vi "InitModuleManager.vi"(8 "error in (no error)":errorcluster, 10 "mmanager":path, 11 "SensorInfos":T3) -> (0 "error out (no error)":errorcluster, 3 "Sensor Engine Datas":T1[](array[typedef]))   [LabVIEW 2023, in "MM.lvlib"]
uses:
  MM.lvlib
  Shared/SensorInfos.ctl
  Shared/SensorInfo.ctl
  Shared/Sensor Name.ctl
  Shared/Protocol.ctl
  MM Data.ctl
  MM Objects.ctl
  MM Object.ctl
  Sensor Engine Data.ctl
  DataContainer/DataContainer.lvclass
  <vilib>/xnet/xnet.llb/XNET Frame FlexRay.ctl
  <vilib>/xnet/xnet.llb/XNET Frame Type FlexRay.ctl
  <vilib>/xnet/xnet.llb/XNET String To IO Name (Signal).vi
  <vilib>/xnet/xnet.llb/XNET Create Session (Conversion).vi
  <resource>/objmgr/xnet.rc
  Shared/Vires VTD Shared.lvlib
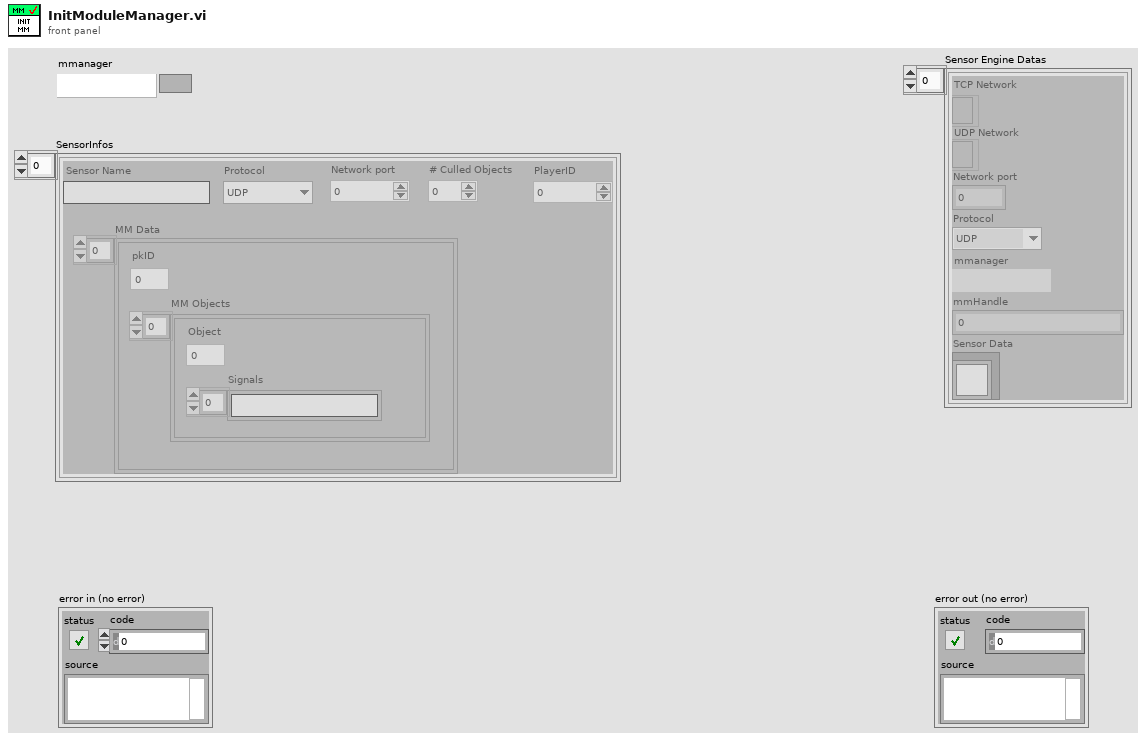
[diagram p1: front panel]
types:
  T1 = typedef "MM.lvlib/Sensor Engine Data.ctl" = cluster{"TCP Network":refnum<k5>, "UDP Network":refnum<k16>, "Network port":i32, "Protocol":T2, "mmanager":path, "mmHandle":u64, "Sensor Data":refnum<class "DataContainer.lvclass">}
  T2 = typedef "Vires VTD Shared.lvlib/Protocol.ctl" = enum16{"UDP", "TCP"}
  T3 = typedef "Vires VTD Shared.lvlib/SensorInfos.ctl" = T4[]
  T4 = typedef "Vires VTD Shared.lvlib/SensorInfo.ctl" = cluster{"Sensor Name":T5, "Protocol":T2, "Network port":i32, "# Culled Objects":i32, "PlayerID":u8, "MM Data":T6}
  T5 = typedef "Vires VTD Shared.lvlib/Sensor Name.ctl" = string
  T6 = typedef "Vires VTD Shared.lvlib/MM Data.ctl" = T7[]
  T7 = typedef "MM.lvlib/MM Objects.ctl" = cluster{"pkID":i32, "MM Objects":T8[]}
  T8 = typedef "MM.lvlib/MM Object.ctl" = cluster{"Object":i32, "Signals":string[]}
  T9 = typedef "XNET Frame FlexRay.ctl" = cluster{"timestamp":timestamp, "payload":u8[], "slot":u16, "type":T10, "cycle count":u8, "startup?":bool, "sync?":bool, "preamble?":bool, "ch A":bool, "ch B":bool, "echo?":bool}
  T10 = typedef "XNET Frame Type FlexRay.ctl" = u8
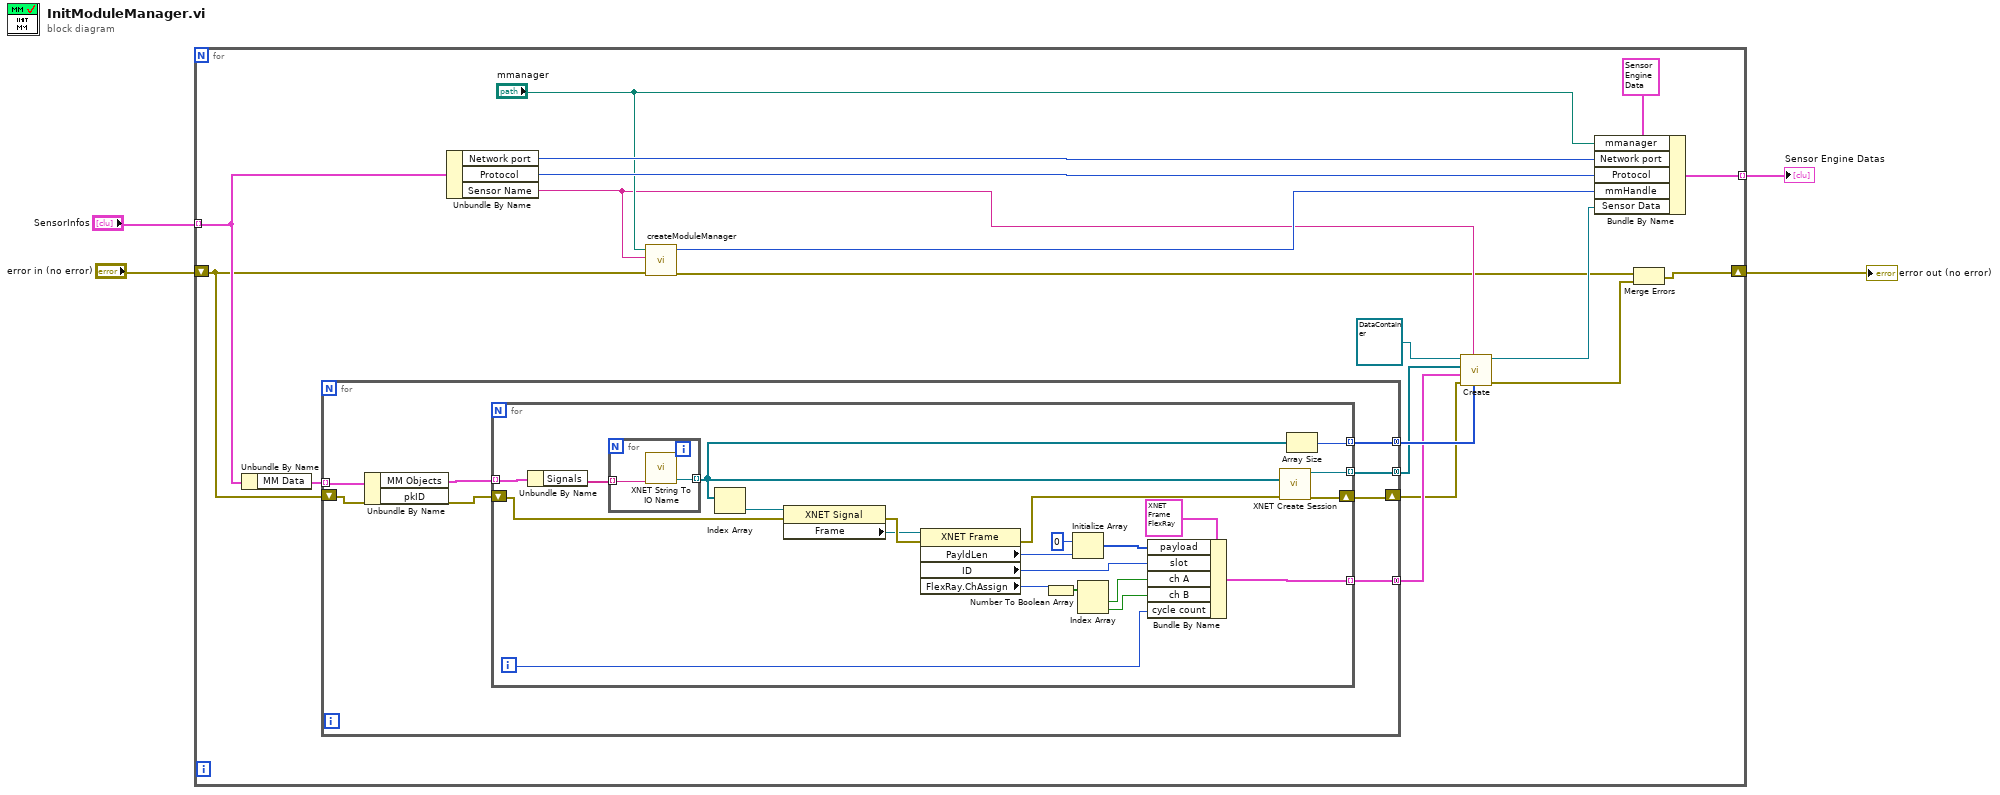
[diagram p0: block diagram]
diagram:
  n1 = for {
    tunnel: "SensorInfos" -> [w23] mode=indexing
    shift-right: [w5] -> w4
    shift-left: "error in (no error)" -> [w9]
    tunnel: [w18] -> w2 mode=indexing
    n2 = Unbundle By Name(w23) -> ("MM Data"=w22:T6)
    n3 = for {
      shift-right: [w30] -> w8
      shift-left: w9 -> [w29]
      tunnel: [w28] -> w12 mode=concatenating
      tunnel: [w27] -> w11 mode=concatenating
      tunnel: w22 -> [w26] mode=indexing
      tunnel: [w24] -> w14 mode=concatenating
      n4 = Unbundle By Name(w26) -> ("MM Objects"=w25:T8[])  [unwired: 1 out]
      n5 = for {
        tunnel: [w39] -> w27 mode=indexing
        tunnel: [w35] -> w28 mode=indexing
        shift-right: [w37] -> w30
        shift-left: w29 -> [w36]
        tunnel: w25 -> [w34] mode=indexing
        tunnel: [w31] -> w24 mode=indexing
        i -> [w33]
        n6 = Unbundle By Name(w34) -> ("Signals"=w52:string[])
        n7 = for {
          tunnel: w52 -> [w54] mode=indexing
          tunnel: [w53] -> w32 mode=indexing
          n8 = call-poly <vilib>:"XNET String To IO Name.vi"("string"=w54) -> ("XNET Signal"=w53:refnum<k21>)  [unwired: 4 out]
        }
        n9 = Index Array(array=w32) -> (element=w40:refnum<k21>)  [unwired: 1 in]
        n10 = property class="XNET Signal"(reference=w40, error in=w36) -> (error out=w51:errorcluster, "Frame"=w50:refnum<k21>)  [unwired: 1 out]
        n11 = property class="XNET Frame"(reference=w50, error in=w51) -> (error out=w38:errorcluster, "PayldLen"=w43:u32, "ID"=w45:u32, "FlexRay.ChAssign"=w46:u32)  [unwired: 1 out]
        n12 = Number To Boolean Array(number=w46) -> (Boolean array=w41:bool[])
        n13 = Initialize Array(u8 0 ("element"), w43) -> (w44:u8[])
        n14 = Index Array(array=w41) -> (element #1=w47:bool, element #2=w48:bool)  [unwired: 2 in]
        n15 = Bundle By Name(cluster=T9 {"timestamp"=timestamp(0 s since 1904-01-01), "payload"=[], "slot"=1, "type"=32, "cycle count"=0, "startup?"=FALSE, "sync?"=FALSE, "preamble?"=FALSE, "ch A"=FALSE, "ch B"=FALSE, "echo?"=FALSE} ("FlexRay frame"), "payload"=w44, "slot"=w45, "ch A"=w47, "ch B"=w48, "cycle count"=w33) -> (w39:T9)
        n16 = call-poly <vilib>:"XNET Create Session.vi"("signal list"=w32, "error in (no error)"=w38) -> ("session out"=w35:refnum<k21>, "error out"=w37:errorcluster)  [unwired: 12 in]
        n17 = Array Size(array=w32) -> (size(s)=w31:i32)
      }
    }
    n18 = Unbundle By Name(w23) -> ("Network port"=w20:i32, "Protocol"=w19:T2, "Sensor Name"=w15:T5)
    n19 = call "createModuleManager.vi"("error in (no error)"=w9, "sensorName"=w15, "path in"="mmanager") -> ("error out"=w7:errorcluster, "mmHandle"=w16:u64)  [unwired: 7 in]
    n20 = call-dynamic "Create.vi"("noSignals"=w14, "Container ID"=w15, "error in (no error)"=w8, "Package Data"=w11, "Conversion References"=w12, "DataContainer in"=refnum<class "DataContainer.lvclass"> refnum) -> ("error out"=w6:errorcluster, "DataContainer out"=w10:refnum<class "DataContainer.lvclass">)  [unwired: 4 in]
    n21 = Bundle By Name(cluster=T1 {"TCP Network"=refnum, "UDP Network"=refnum, "Network port"=0, "Protocol"=enum."UDP", "mmanager"=path "", "mmHandle"=0, "Sensor Data"=refnum} ("MM.lvlib:Sensor Engine Data"), "mmanager"="mmanager", "Network port"=w20, "Protocol"=w19, "mmHandle"=w16, "Sensor Data"=w10) -> (w18:T1)
    n22 = Merge Errors(w7, w6) -> (w5:errorcluster)
  }
  "error out (no error)" <- w4
  "Sensor Engine Datas" <- w2
